vi "py2vi-lvcli.vi"(11 "Args":string[](array[string])) -> (2 "Output":string, 3 "Output Code":i32)   [LabVIEW 2026]
uses:
  Actors/File Logger/File Logger/File Logger.lvclass
  C:/Program Files/National Instruments/LabVIEW 2026/vi.lib/ActorFramework/Actor/Actor.lvclass
  Actors/Runner/Runner/Runner.lvclass
  Actors/File Logger/File Logger/File Logger.lvclass/File Logger.ctl
  Actors/Runner/Runner/Runner.lvclass/Runner.ctl
  Interfaces/ILogger Client/ILogger Client Messages/Set Logger Enqueuer Msg/Set Logger Enqueuer Msg.lvclass/Set Logger Enqueuer Msg.ctl
  <vilib>/ActorFramework/Message Enqueuer/Message Enqueuer.lvclass/Message Enqueuer.ctl
  Interfaces/IRunner/IRunner Messages/Set Interfaces Msg/Set Interfaces Msg.lvclass/Set Interfaces Msg.ctl
  Interfaces/IRunner/IRunner Messages/Run Msg/Run Msg.lvclass/Run Msg.ctl
  <vilib>/ActorFramework/Stop Msg/Stop Msg.lvclass/Stop Msg.ctl
  Actors/Runner/Runner/Write Stop Event.vi
  Actors/File Logger/File Logger/Write Log File.vi
  <vilib>/ActorFramework/Message Enqueuer/Enqueue.vi
  <vilib>/ActorFramework/Message Enqueuer/Enqueue Critical.vi
  Interfaces/ILogger Client/ILogger Client Messages/Set Logger Enqueuer Msg/Set Logger Enqueuer Msg.lvclass
  C:/Program Files/National Instruments/LabVIEW 2026/vi.lib/ActorFramework/Message/Message.lvclass
  Interfaces/IRunner/IRunner Messages/Set Interfaces Msg/Set Interfaces Msg.lvclass
  Interfaces/IRunner/IRunner Messages/Run Msg/Run Msg.lvclass
  <vilib>/ActorFramework/Stop Msg/Stop Msg.lvclass
  <vilib>/ActorFramework/Message Priority Queue/Priority Enqueue.vi
  <vilib>/ActorFramework/Actor/Actor.lvclass
panel:
  # "py2vi Launcher for LabVIEWCLI"
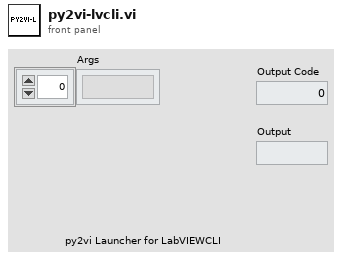
[diagram p1: front panel]
types:
  T1 = typedef "NI_App_Builder_API.lvlib/Build Specification Version.ctl" = cluster{"Major":u16, "Minor":u16, "Fix":u16, "Build":u16}
  T2 = typedef "IRunner.lvlib/IRunner.lvclass/Interfaces--cluster.ctl" = cluster{"IProject Manager":refnum<class "IProject Manager.lvclass">, "IFile Manager":refnum<class "IFile Manager.lvclass">, "IPython Caller":refnum<class "IPython Caller.lvclass">, "IElement Manager":refnum<class "IElement Manager.lvclass">, "ILV File Creator":refnum<class "ILV File Creator.lvclass">, "IHash Whitelist Handler":refnum<class "IHash Whitelist Handler.lvclass">}
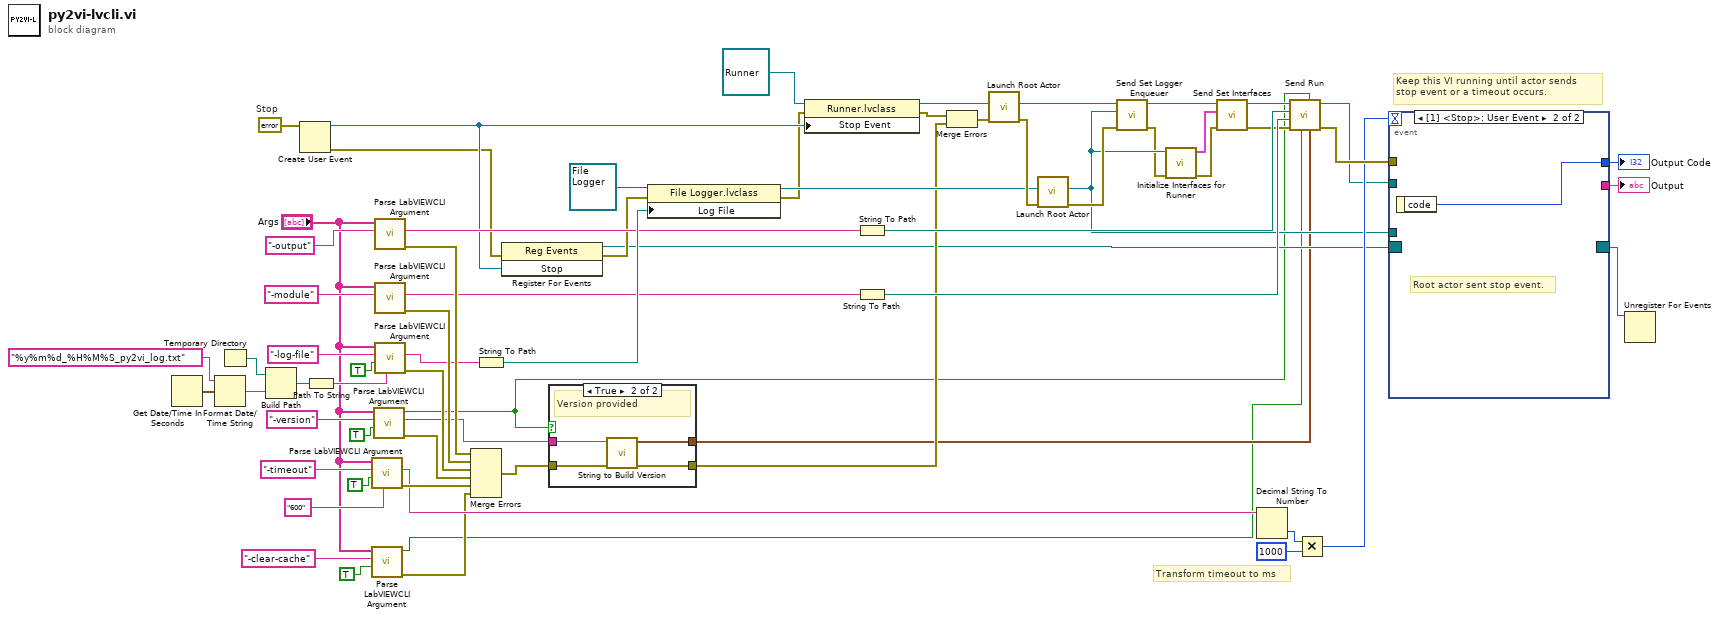
[diagram p0: block diagram]
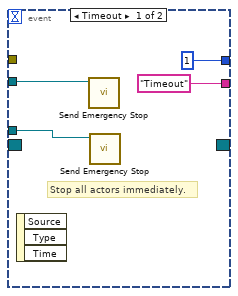
[diagram p2: hidden frame]
diagram:
  w1 = errorcluster {"status"=FALSE, "code"=0, "source"=""}  # Stop
  # "Transform timeout to ms"
  # "Keep this VI running until actor sends stop event or a timeout occurs."
  n1 = Get Date/Time In Seconds() -> (seconds since 1Jan1904=w36:timestamp)
  n2 = Format Date/Time String(time format string (%c)="%y%m%d_%H%M%S_py2vi_log.txt", seconds (now)=w36) -> (date/time string=w33:string)  [unwired: 1 in]
  n3 = Temporary Directory() -> (w34:path)
  n4 = Build Path(base path=w34, name or relative path=w33) -> (appended path=w32:path)
  n5 = Create User Event(user event datatype=w1) -> (user event=w29:refnum<user-event>, error out=w28:errorcluster)  [unwired: 1 in]
  n6 = Path To String(path=w32) -> (string=w31:string)
  n7 = call "Parse LabVIEWCLI Argument.vi"("Default"="600", "Optional"=TRUE, "Identifier"="-timeout" ("Option Key"), "Args"="Args") -> ("error out"=w30:errorcluster, "Value"=w21:string)  [unwired: 5 in, 1 out]
  n8 = call "Parse LabVIEWCLI Argument.vi"("Optional"=TRUE, "Identifier"="-clear-cache" ("Option Key"), "Args"="Args") -> ("error out"=w5:errorcluster, "Found"=w3:bool)  [unwired: 6 in, 1 out]
  n9 = call "Parse LabVIEWCLI Argument.vi"("Optional"=TRUE, "Identifier"="-version" ("Option Key"), "Args"="Args") -> ("error out"=w51:errorcluster, "Value"=w45:string, "Found"=w2:bool)  [unwired: 6 in]
  n10 = call "Parse LabVIEWCLI Argument.vi"("Identifier"="-output" ("Option Key"), "Args"="Args") -> ("error out"=w52:errorcluster, "Value"=w41:string)  [unwired: 7 in, 1 out]
  n11 = call "Parse LabVIEWCLI Argument.vi"("Identifier"="-module" ("Option Key"), "Args"="Args") -> ("error out"=w49:errorcluster, "Value"=w40:string)  [unwired: 7 in, 1 out]
  n12 = call "Parse LabVIEWCLI Argument.vi"("Default"=w31, "Optional"=TRUE, "Identifier"="-log-file" ("Option Key"), "Args"="Args") -> ("error out"=w50:errorcluster, "Value"=w48:string)  [unwired: 5 in, 1 out]
  n13 = Merge Errors(w52, w49, w50, w51, w30, w5) -> (w44:errorcluster)
  n14 = String To Path(string=w48) -> (path=w46:path)
  n15 = register-events(error in=w28, w29) -> (reference out=w16:refnum<event-registration>, error out=w27:errorcluster)  [unwired: 1 in]
  n16 = case shown="True" w2 {
    tunnel: w45 -> [_ w72]
    tunnel: [_ w71] -> w4
    tunnel: w44 -> [w68 w70]
    tunnel: [w68 w69] -> w42
    frame False {
      # "No version provided."
    }
    frame True {
      # "Version provided"
      n17 = call "String to Build Version.vi"("error in"=w70, "Version String"=w72) -> ("error out"=w69:errorcluster, "Build Specification Version"=w71:T1)  [unwired: 8 in]
    }
  }
  n18 = property class="File Logger.lvclass"(reference=refnum<class "File Logger.lvclass"> refnum ("File Logger.lvlib:File Logger.lvclass"), error in=w27, "Log File"=w46) -> (reference out=w43:refnum<class "File Logger.lvclass">, error out=w26:errorcluster)
  n19 = property class="Runner.lvclass"(reference=refnum<class "Runner.lvclass"> refnum ("G-CLI Runner.lvlib:G-CLI Runner.lvclass"), error in=w26, "Stop Event"=w29) -> (reference out=w66:refnum<class "Runner.lvclass">, error out=w24:errorcluster)
  n20 = String To Path(string=w41) -> (path=w64:path)
  n21 = String To Path(string=w40) -> (path=w63:path)
  n22 = Merge Errors(w24, w42) -> (w25:errorcluster)
  n23 = call <vilib>:"Launch Root Actor.vi"("error in (no error)"=w25, "Actor"=w66) -> ("error out"=w61:errorcluster, "Actor's Enqueuer"=w62:refnum<class "Message Enqueuer.lvclass">)  [unwired: 8 in]
  n24 = call <vilib>:"Launch Root Actor.vi"("error in (no error)"=w61, "Actor"=w43) -> ("error out"=w65:errorcluster, "Actor's Enqueuer"=w13:refnum<class "Message Enqueuer.lvclass">)  [unwired: 8 in]
  n25 = call "Send Set Logger Enqueuer.vi"("error in (no error)"=w65, "Logger"=w13, "Message Enqueuer"=w62) -> ("error out"=w12:errorcluster, "Message Enqueuer out"=w10:refnum<class "Message Enqueuer.lvclass">)  [unwired: 7 in]
  n26 = call "Initialize Interfaces for Runner.vi"("error in"=w12, "Logger Enqueuer"=w13) -> ("error out"=w9:errorcluster, "Interfaces"=w11:T2)  [unwired: 8 in]
  n27 = call "Send Set Interfaces.vi"("error in (no error)"=w9, "Interfaces"=w11, "Message Enqueuer"=w10) -> ("error out"=w59:errorcluster, "Message Enqueuer out"=w60:refnum<class "Message Enqueuer.lvclass">)  [unwired: 7 in]
  n28 = Decimal String To Number(string=w21) -> (number=w20:i32)  [unwired: 2 in, 1 out]
  n29 = call "Send Run.vi"("Build Specification Version"=w4, "Set PPL Version"=w2, "Clear Compiled Object Cache"=w3, "error in (no error)"=w59, "Python Module"=w63, "Output Folder"=w64, "Message Enqueuer"=w60) -> ("error out"=w22:errorcluster, "Message Enqueuer out"=w17:refnum<class "Message Enqueuer.lvclass">)  [unwired: 3 in]
  n30 = Multiply(x=w20, y=1000) -> (x*y=w18:i32)
  n31 = event shown="[1] <Stop>: User Event" {
    selector: w16 -> [_ _]
    dyn-events: [_ _] -> w23
    timeout: w18 -> [_ _]
    tunnel: w17 -> [w76 _]
    tunnel: w13 -> [w75 _]
    tunnel: w22 -> [_ _]
    tunnel: [1 w77] -> w15
    tunnel: ["Timeout" _] -> w14
    event Timeout {
      # "Stop all actors immediately."
      n32 = event-data() -> ()  [unwired: 1 in, 3 out]
      n33 = call <vilib>:"Send Emergency Stop.vi"("Message Enqueuer"=w76) -> ()  [unwired: 10 in, 1 out]
      n34 = call <vilib>:"Send Emergency Stop.vi"("Message Enqueuer"=w75) -> ()  [unwired: 10 in, 1 out]
    }
    event User Event {
      # "Root actor sent stop event."
      n35 = event-data() -> ("code"=w77:i32)  [unwired: 1 in]
    }
  }
  "Output Code" <- w15
  "Output" <- w14
  n36 = Unregister For Events(event registration refnum=w23) -> ()  [unwired: 1 in, 1 out]
